vi "Get Package Attributes (All Versions).vi"(8 "error in":errorcluster, 11 "package name":string) -> (0 "error out":errorcluster, 2 "package attributes (all versions)":T1[](array[typedef]), 3 "package name out":string)   [LabVIEW 2014, in "NIPM_API.lvlib"]
doc: "Returns the attributes for all versions of the specified package\n\nINPUT(s)\n<B>Package name</B>: Specifies the package\n\nOUTPUT(s)\n<B>Package name out</B>: Outputs the package name\n\n<B>Package attributes (all versions)</B>: Outputs a 1D array containing the package attributes for all versions of the specified package\n\nDETAILS:\nThis VI checks for package attribute data in both installed packages and packages in registered feeds."
uses:
  NIPM_API.lvlib
  _support/package attributes.ctl
panel:
  out "cmd standard output (info-installed)":string
  out "cmd standard output (info)":string
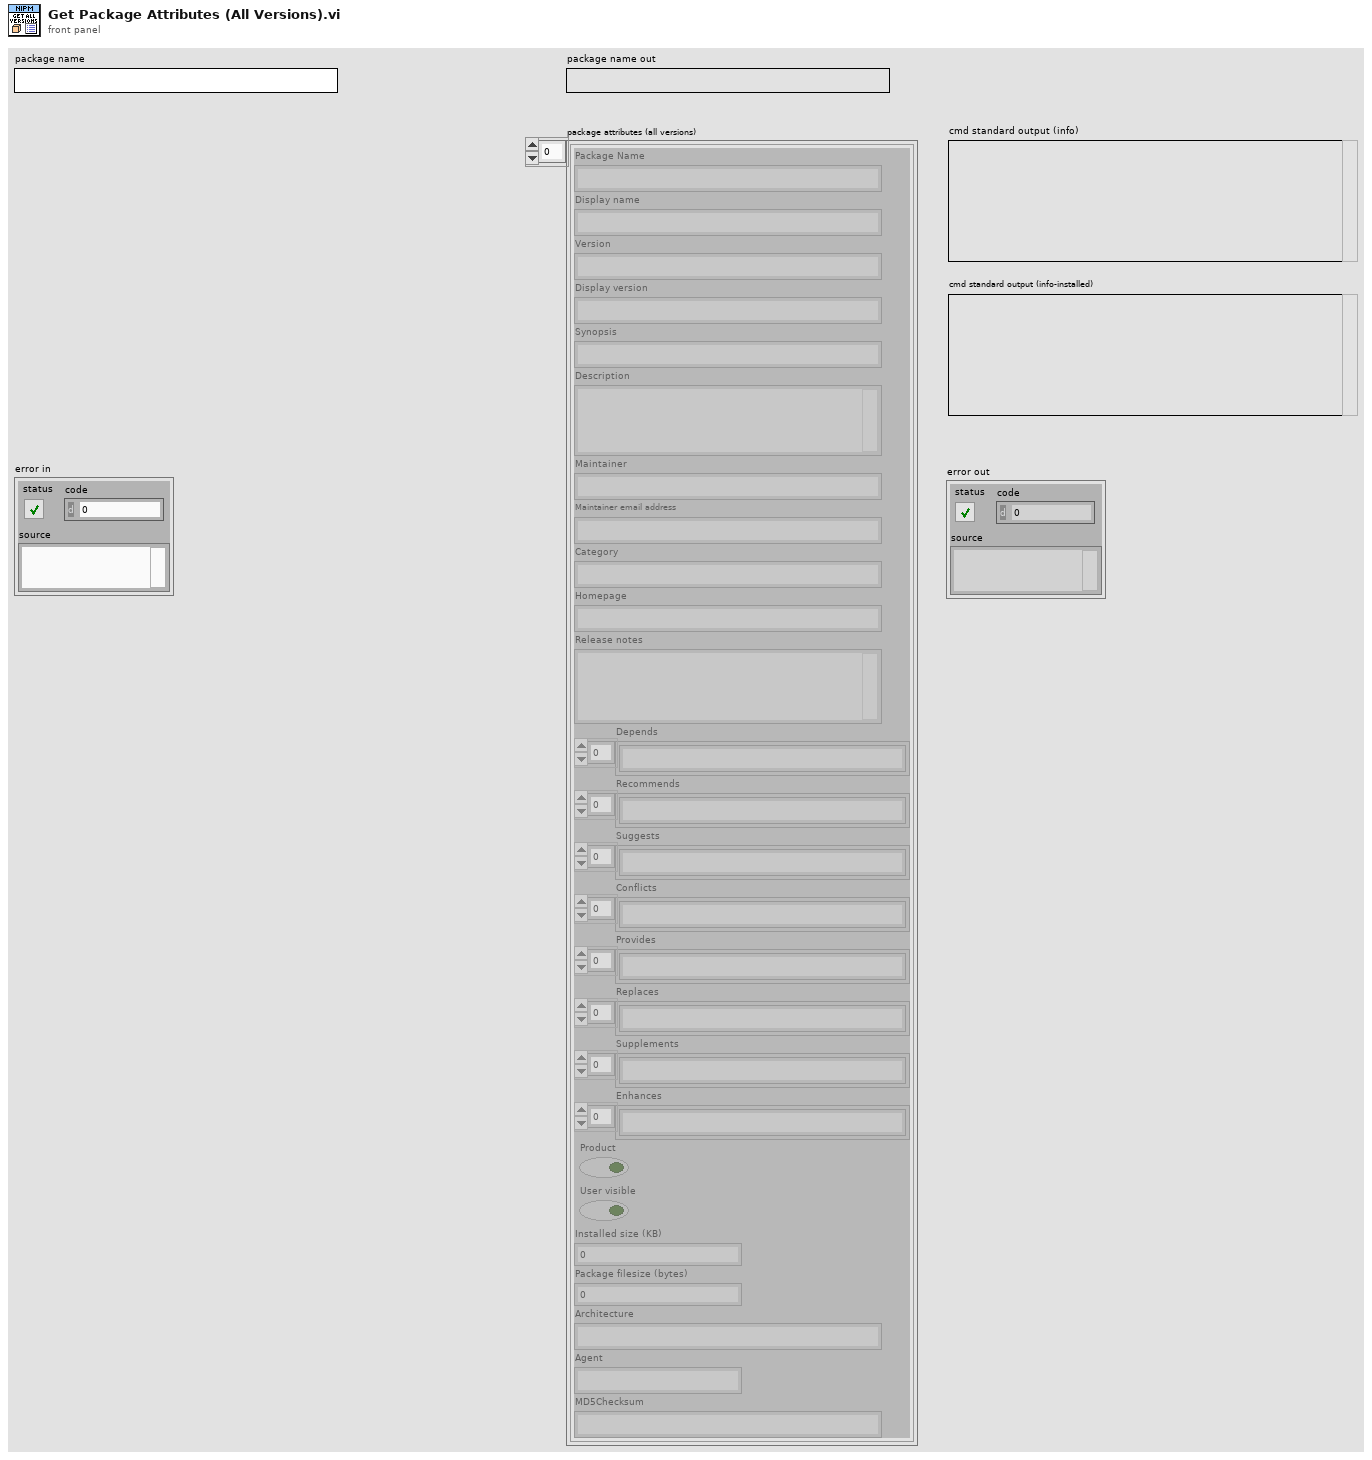
[diagram p1: front panel]
types:
  T1 = typedef "NIPM_API.lvlib/package attributes.ctl" = cluster{"Package Name":string, "Display name":string, "Version":string, "Display version":string, "Synopsis":string, "Description":string, "Maintainer":string, "Maintainer email address":string, "Category":string, "Homepage":string, "Release notes":string, "Depends":string[], "Recommends":string[], "Suggests":string[], "Conflicts":string[], "Provides":string[], "Replaces":string[], "Supplements":string[], "Enhances":string[], "Product":bool, "User visible":bool, "Installed size (KB)":u64, "Package filesize (bytes)":u64, "Architecture":string, "Agent":string, "MD5Checksum":string}
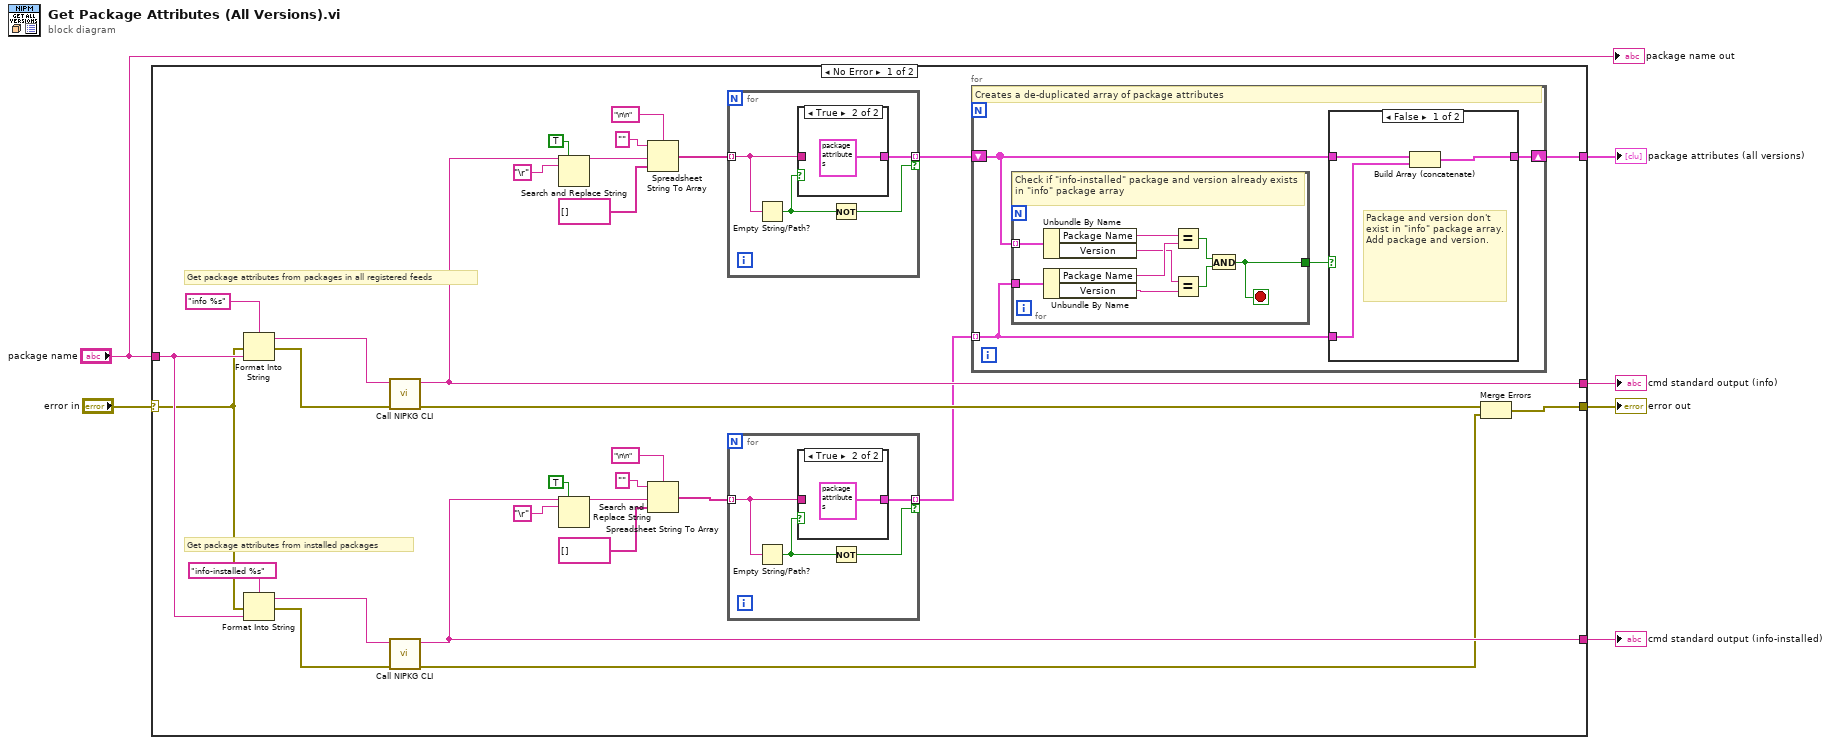
[diagram p0: block diagram]
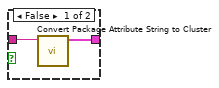
[diagram p3: hidden frame]
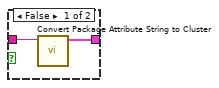
[diagram p4: hidden frame]
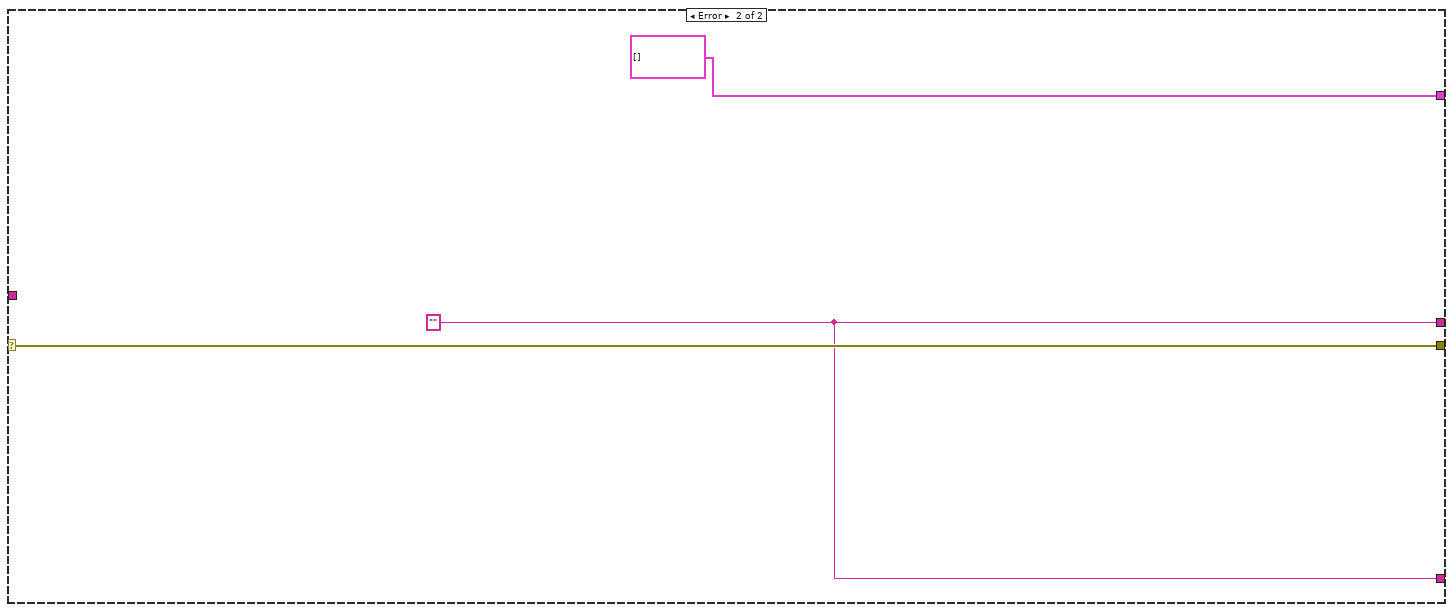
[diagram p5: hidden frame]
diagram:
  n1 = case shown="No Error" "error in" {
    selector: "error in" -> [w13 w70]
    tunnel: [w8 w70] -> w5
    tunnel: [w32 w68] -> w4
    tunnel: "package name" -> [w14 _]
    tunnel: [w9 T1[] []] -> w2
    tunnel: [w12 w68] -> w1
    frame No Error {
      # "Get package attributes from installed packages"
      # "Get package attributes from packages in all registered feeds"
      n2 = Format Into String(format string="info %s", error in=w13, w14) -> (resulting string=w33:string, error out=w35:errorcluster)  [unwired: 1 in]
      n3 = Format Into String(format string="info-installed %s", error in=w13, w14) -> (resulting string=w17:string, error out=w16:errorcluster)  [unwired: 1 in]
      n4 = call "Call NIPKG CLI.vi"("error in (no error)"=w35, "command"=w33) -> ("error out"=w34:errorcluster, "command line standard output"=w32:string)  [unwired: 8 in]
      n5 = call "Call NIPKG CLI.vi"("error in (no error)"=w16, "command"=w17) -> ("error out"=w7:errorcluster, "command line standard output"=w12:string)  [unwired: 8 in]
      n6 = Search and Replace String(replace all?=TRUE ("replace all? (F)"), input string=w32, search string="\r") -> (result string=w29:string)  [unwired: 5 in, 3 out]
      n7 = Search and Replace String(replace all?=TRUE ("replace all? (F)"), input string=w12, search string="\r") -> (result string=w20:string)  [unwired: 5 in, 3 out]
      n8 = Spreadsheet String To Array(delimiter (Tab)="\n\n", format string="", spreadsheet string=w29, array type (2D Dbl)=string[] []) -> (array=w25:string[])
      n9 = Spreadsheet String To Array(delimiter (Tab)="\n\n", format string="", spreadsheet string=w20, array type (2D Dbl)=string[] []) -> (array=w24:string[])
      n10 = for {
        tunnel: w25 -> [w63] mode=indexing
        tunnel: [w64] -> w10 mode=indexing if=w61
        n11 = Empty String/Path?(string/path=w63) -> (empty?=w62:bool)
        n12 = case shown="True" w62 {
          tunnel: [w66 T1 {"Package Name"="", "Display name"="", "Version"="", "Display version"="", "Synopsis"="", "Description"="", "Maintainer"="", "Maintainer email address"="", "Category"="", "Homepage"="", "Release notes"="", "Depends"=[], "Recommends"=[], "Suggests"=[], "Conflicts"=[], "Provides"=[], "Replaces"=[], "Supplements"=[], "Enhances"=[], "Product"=FALSE, "User visible"=FALSE, "Installed size (KB)"=0, "Package filesize (bytes)"=0, "Architecture"="", "Agent"="", "MD5Checksum"=""} ("package attributes")] -> w64
          tunnel: w63 -> [w65 _]
          frame False {
            n13 = call "Convert Package Attribute String to Cluster.vi"("package attributes string"=w65) -> ("package attributes"=w66:T1)  [unwired: 9 in, 1 out]
          }
          frame True {
          }
        }
        n14 = Not(x=w62) -> (.not. x?=w61:bool)
      }
      n15 = for {
        tunnel: w24 -> [w56] mode=indexing
        tunnel: [w57] -> w11 mode=indexing if=w54
        n16 = Empty String/Path?(string/path=w56) -> (empty?=w55:bool)
        n17 = case shown="True" w55 {
          tunnel: [w59 T1 {"Package Name"="", "Display name"="", "Version"="", "Display version"="", "Synopsis"="", "Description"="", "Maintainer"="", "Maintainer email address"="", "Category"="", "Homepage"="", "Release notes"="", "Depends"=[], "Recommends"=[], "Suggests"=[], "Conflicts"=[], "Provides"=[], "Replaces"=[], "Supplements"=[], "Enhances"=[], "Product"=FALSE, "User visible"=FALSE, "Installed size (KB)"=0, "Package filesize (bytes)"=0, "Architecture"="", "Agent"="", "MD5Checksum"=""} ("package attributes")] -> w57
          tunnel: w56 -> [w58 _]
          frame False {
            n18 = call "Convert Package Attribute String to Cluster.vi"("package attributes string"=w58) -> ("package attributes"=w59:T1)  [unwired: 9 in, 1 out]
          }
          frame True {
          }
        }
        n19 = Not(x=w55) -> (.not. x?=w54:bool)
      }
      n20 = for {
        tunnel: w11 -> [w38] mode=indexing
        shift-right: [w37] -> w9
        shift-left: w10 -> [w40]
        # "Creates a de-duplicated array of package attributes"
        n21 = for {
          tunnel: w40 -> [w46] mode=indexing
          tunnel: w38 -> [w53]
          tunnel: [w45] -> w39
          stop <- w45 stop-if-true
          # "Check if \"info-installed\" package and version already exists in \"info\" package array"
          n22 = Unbundle By Name(w46) -> ("Package Name"=w52:string, "Version"=w50:string)
          n23 = Unbundle By Name(w53) -> ("Package Name"=w51:string, "Version"=w49:string)
          n24 = Equal?(x=w52, y=w51) -> (x = y?=w48:bool)
          n25 = Equal?(x=w50, y=w49) -> (x = y?=w47:bool)
          n26 = And(x=w48, y=w47) -> (x .and. y?=w45:bool)
        }
        n27 = case shown="False" w39 {
          tunnel: w40 -> [w43 w44]
          tunnel: w38 -> [w42 _]
          tunnel: [w41 w44] -> w37
          frame False {
            # "Package and version don't exist in \"info\" package array.  Add package and version."
            n28 = Build Array (concatenate)(w43, w42) -> (w41:T1[])
          }
          frame True {
            # "Package and version already exist in \"info\" package array.  Do not add package and version."
          }
        }
      }
      n29 = Merge Errors(w34, w7) -> (w8:errorcluster)
    }
    frame Error {
      w68 = "" ("standard output")
    }
  }
  "error out" <- w5
  "cmd standard output (info)" <- w4
  "package attributes (all versions)" <- w2
  "cmd standard output (info-installed)" <- w1
  "package name out" <- "package name"
